vi "Parse Common Prefixes.vi"(8 "error in (no error)":errorcluster, 11 "Response body":string) -> (0 "error out":errorcluster, 3 "Common Prefixes":string[](array[string]))   [LabVIEW 2015, in "NI_AWS_S3.lvlib" / "Object.lvlib"]
doc: "Parse out the CommonPrefixes part of the Response body of a List bucket request."
uses:
  Object.lvlib
  XML Parsing/NI_XML Parsing.lvlib
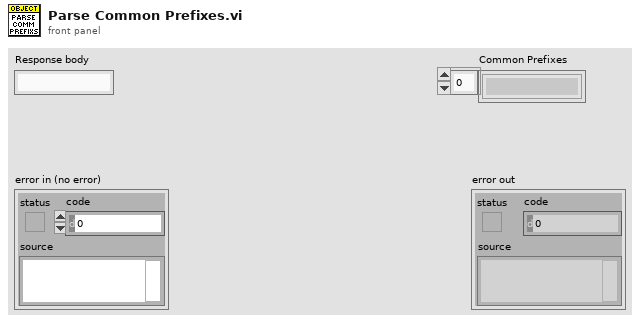
[diagram p1: front panel]
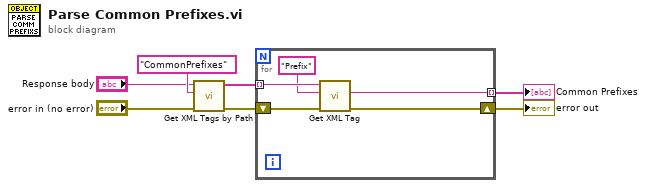
[diagram p0: block diagram]
diagram:
  n1 = call "Get XML Tags by Path.vi"("error in (no error)"="error in (no error)", "Tag path"="CommonPrefixes", "XML String in"="Response body") -> ("error out"=w5:errorcluster, "Matching tag values"=w6:string[])  [unwired: 7 in]
  n2 = for {
    tunnel: w6 -> [w11] mode=indexing
    shift-right: [w9] -> w2
    shift-left: w5 -> [w12]
    tunnel: [w8] -> w1 mode=indexing
    n3 = call "Get XML Tag.vi"("error in (no error)"=w12, "Tag name"="Prefix" ("Tag path"), "XML String in"=w11) -> ("error out"=w9:errorcluster, "Tag value"=w8:string)  [unwired: 4 in, 3 out]
  }
  "Common Prefixes" <- w1
  "error out" <- w2
